vi "Read Boolean Control Value.vi"(8 "error in (no error)":errorcluster, 11 "Boolean in":refnum<vi>) -> (0 "error out":errorcluster, 3 "boolean value out":bool)   [LabVIEW 2021]
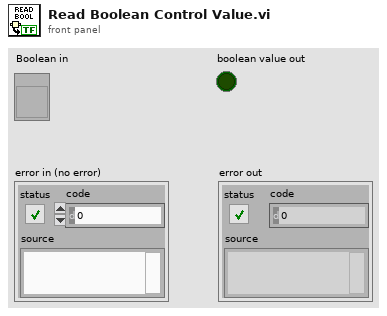
[diagram p1: front panel]
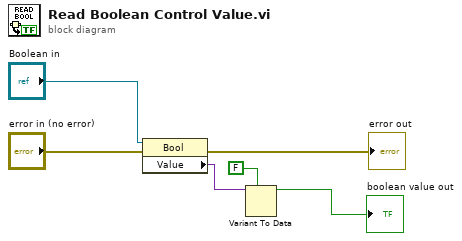
[diagram p0: block diagram]
diagram:
  n1 = property class="Bool"(reference="Boolean in", error in="error in (no error)") -> (error out=→"error out":errorcluster, "Value"=w5:variant)  [unwired: 1 out]
  n2 = Variant To Data(type=FALSE, Variant=w5) -> (data=→"boolean value out":bool)  [unwired: 1 in, 1 out]
